vi "Get All Test Registrations.vi"(8 "error in (no error)":errorcluster, 11 "Test Event Storage in":refnum<class "Test Event Storage.lvclass">) -> (0 "error out":errorcluster, 1 "Test Registrations":T1[](array[typedef]), 2 "Test IDs":string[](array[string]), 3 "Test Event Storage out":refnum<class "Test Event Storage.lvclass">, 5 "Test Parent IDs":string[](array[string]))   [LabVIEW 2020, in "Caraya.lvlib" / "Test Event Storage.lvclass"]
uses:
  Test Event Storage.lvclass
  Test Result/Test Node (Extended).ctl
  Test Result/Test Registration Data.ctl
  Test Event Storage.lvclass/Test Event Storage.ctl
  test store -- cluster.ctl
  Test Manager Message Test/TestManagerMsg.Test.lvclass
  Test Result/Test Result.lvclass
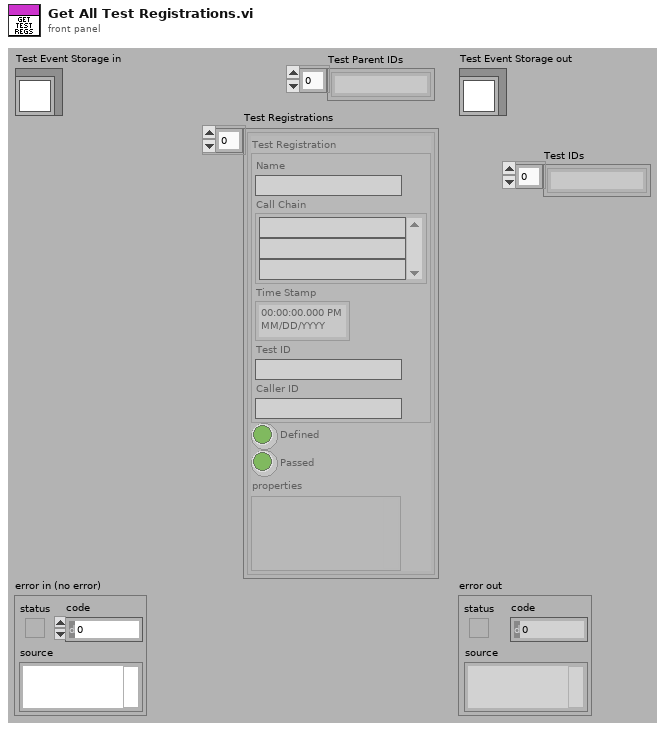
[diagram p1: front panel]
types:
  T1 = typedef "Caraya.lvlib/Test Result.lvclass/Test Node (Extended).ctl" = cluster{"Test Registration":T2, "Defined":bool, "Passed":bool, "properties":variant}
  T2 = typedef "Caraya.lvlib/Test Result.lvclass/Test Registration Data.ctl" = cluster{"Name":string, "Call Chain":string[], "Time Stamp":timestamp, "Test ID":string, "Caller ID":string}
  T3 = typedef "Caraya.lvlib/Test Event Storage.lvclass/test store -- cluster.ctl" = cluster{"Test":refnum<class "TestManagerMsg.Test.lvclass">, "Defined":bool, "Passed":bool, "properties":variant, "assert-ids":variant}
  T4 = cluster{i32, "Time Stamp":timestamp, "Caller ID":string, "Test ID":string, "Test Node 2":T1}
  T5 = cluster{i32, "Time Stamp":timestamp, "Caller ID":string, "Test ID":string, "Test Node 2":T1}[]
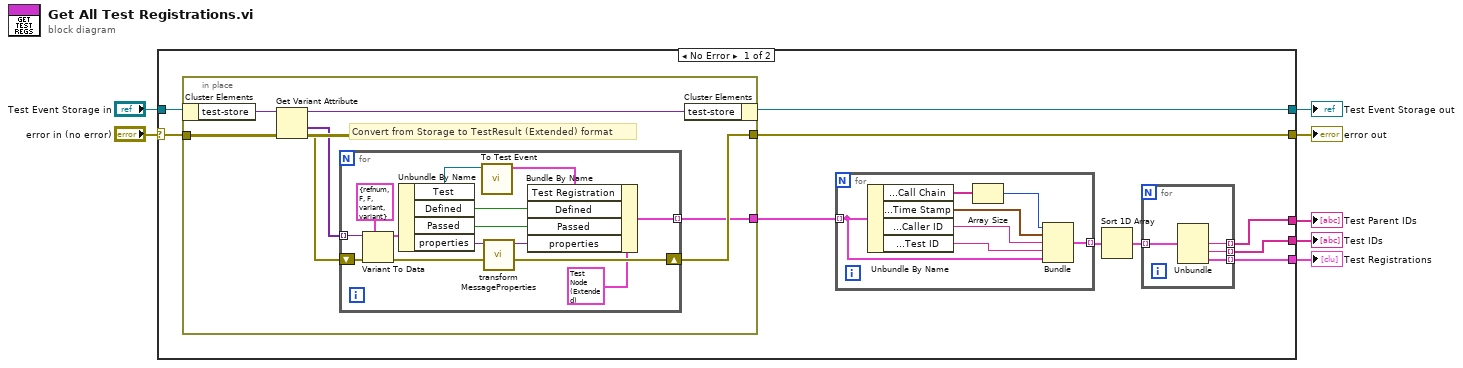
[diagram p0: block diagram]
diagram:
  n1 = case shown="No Error" "error in (no error)" {
    selector: "error in (no error)" -> [w17 w50]
    tunnel: [w10 w50] -> w6
    tunnel: [w9 w49] -> w4
    tunnel: "Test Event Storage in" -> [w8 w49]
    tunnel: [w13 _] -> w3
    tunnel: [w12 _] -> w2
    tunnel: [w11 _] -> w1
    frame No Error {
      n2 = in-place {
        in-place-border: w17 -> [w23]
        in-place-border: [w19] -> w10
        in-place-border: [w18] -> w16
        # "Convert from Storage to TestResult (Extended) format"
        n3 = in-place-cluster #1(w8) -> ("test-store"=w24:variant)
        n4 = Get Variant Attribute(Variant=w24, error in=w23) -> (duplicate Variant=w22:variant, values=w21:variant[], error out=w20:errorcluster)  [unwired: 2 in, 1 out]
        n5 = for {
          tunnel: w21 -> [w37] mode=indexing
          shift-right: [w35] -> w19
          shift-left: w20 -> [w36]
          tunnel: [w32] -> w18 mode=indexing
          n6 = Variant To Data(error in=w36, type=T3 {"Test"=refnum, "Defined"=FALSE, "Passed"=FALSE, "properties"=variant, "assert-ids"=variant} ("test-store"), Variant=w37) -> (data=w34:T3, error out=w35:errorcluster)
          n7 = Unbundle By Name(w34) -> ("Test"=w28:refnum<class "TestManagerMsg.Test.lvclass">, "Defined"=w31:bool, "Passed"=w30:bool, "properties"=w26:variant)
          n8 = call "To Test Event.vi"("TestManagerMsg.Test in"=w28) -> ("Test Registration"=w29:T2)  [unwired: 10 in]
          n9 = call "transform MessageProperties.vi"("properties (KVP)"=w26) -> ("properties (Variant Attr)"=w25:variant)  [unwired: 10 in]
          n10 = Bundle By Name(cluster=T1 {"Test Registration"={"Name"="", "Call Chain"=[], "Time Stamp"=timestamp(0 s since 1904-01-01), "Test ID"="", "Caller ID"=""}, "Defined"=FALSE, "Passed"=FALSE, "properties"=variant} ("Test Node 2"), "Test Registration"=w29, "Defined"=w31, "Passed"=w30, "properties"=w25) -> (w32:T1)
        }
        n11 = in-place-cluster #1("test-store"=w22) -> (w9:refnum<class "Test Event Storage.lvclass">)
      }
      n12 = for {
        tunnel: w16 -> [w45] mode=indexing
        tunnel: [w48] -> w15 mode=indexing
        n13 = Unbundle By Name(w45) -> ("Test Registration.Call Chain"=w47:string[], "Test Registration.Time Stamp"=w44:timestamp, "Test Registration.Caller ID"=w43:string, "Test Registration.Test ID"=w42:string)
        n14 = Array Size(array=w47) -> (size(s)=w46:i32)
        n15 = Bundle(w46, "Time Stamp"=w44, "Caller ID"=w43, "Test ID"=w42, "Test Node 2"=w45) -> (w48:T4)  [unwired: 1 in]
      }
      n16 = Sort 1D Array(array=w15) -> (sorted array=w14:T5)
      n17 = for {
        tunnel: w14 -> [w41] mode=indexing
        tunnel: [w40] -> w13 mode=indexing
        tunnel: [w39] -> w11 mode=indexing
        tunnel: [w38] -> w12 mode=indexing
        n18 = Unbundle(w41) -> ("Caller ID"=w38:string, "Test ID"=w39:string, "Test Node 2"=w40:T1)  [unwired: 2 out]
      }
    }
    frame Error {
    }
  }
  "error out" <- w6
  "Test Event Storage out" <- w4
  "Test Registrations" <- w3
  "Test Parent IDs" <- w2
  "Test IDs" <- w1
